vi "Display Data.vi"(8 "error in (no error)":errorcluster, 11 "XY Plot":refnum<vi>) -> (0 "error out":errorcluster, 3 "XY Plot out":refnum<vi>)   [LabVIEW 2025, in "Flow Grind.lvlib" / "4way Lap.lvclass"]
uses:
  4way Lap.lvclass
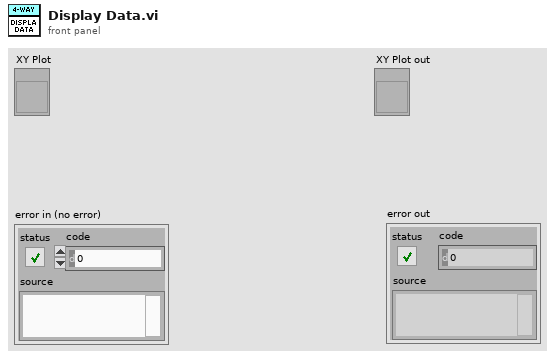
[diagram p1: front panel]
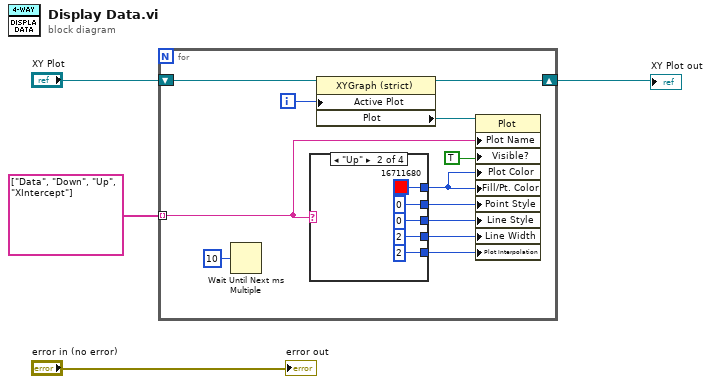
[diagram p0: block diagram]
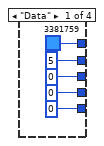
[diagram p2: hidden frame]
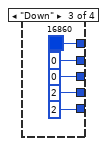
[diagram p3: hidden frame]
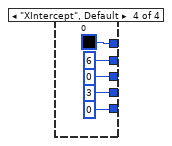
[diagram p4: hidden frame]
diagram:
  n1 = for {
    tunnel: string[] ["Data", "Down", "Up", "XIntercept"] -> [w9] mode=indexing
    shift-right: [w5] -> w1
    shift-left: "XY Plot" -> [w11]
    i -> [w6]
    n2 = Wait Until Next ms Multiple(millisecond multiple=u32 10) -> ()  [unwired: 1 out]
    n3 = case shown="\"Up\"" w9 {
      tunnel: [u32 3381759 ("Plot.Plot Color") u32 16711680 ("Plot.Plot Color") u32 16860 ("Plot.Plot Color") u32 0 ("Plot.Plot Color")] -> w12
      tunnel: [u8 5 ("Plot.Point Style") u8 0 ("Plot.Point Style") u8 0 ("Plot.Point Style") u8 6 ("Plot.Point Style")] -> w16
      tunnel: [u8 0 ("Plot.Line Style") u8 0 ("Plot.Line Style") u8 0 ("Plot.Line Style") u8 0 ("Plot.Line Style")] -> w15
      tunnel: [u8 0 ("Plot.Line Width") u8 2 ("Plot.Line Width") u8 2 ("Plot.Line Width") u8 3 ("Plot.Line Width")] -> w14
      tunnel: [u8 0 ("Plot Interpolation") u8 2 ("Plot Interpolation") u8 2 ("Plot Interpolation") u8 0 ("Plot Interpolation")] -> w13
      frame "Data" {
      }
      frame "Up" {
      }
      frame "Down" {
      }
      frame "XIntercept", Default {
      }
    }
    n4 = property class="XYGraph (strict)"(reference=w11, "Active Plot"=w6) -> (reference out=w5:refnum<vi>, "Plot"=w7:refnum<vi>)  [unwired: 1 in, 1 out]
    n5 = property class="Plot"(reference=w7, "Plot Name"=w9, "Visible?"=TRUE ("Visible"), "Plot Color"=w12, "Fill/Pt. Color"=w12, "Point Style"=w16, "Line Style"=w15, "Line Width"=w14, "Plot Interpolation"=w13) -> ()  [unwired: 1 in, 2 out]
  }
  "XY Plot out" <- w1
  "error out" <- "error in (no error)"
